vi "Prepare.vi"(8 "error in (no error)":errorcluster, 10 "Arguments":T1[](array[typedef]) {"Number" items=["? One or none"=0, "* Any"=-1, "+ At least one"=-2]}, 11 "LV Argument Parser in":refnum<class "LV Argument Parser.lvclass">) -> (0 "error out":errorcluster, 3 "LV Argument Parser out":refnum<class "LV Argument Parser.lvclass">)   [LabVIEW 2020, in "LV ArgParse.lvlib" / "LV Argument Parser.lvclass"]
uses:
  LV Argument Parser.lvclass
  Argument Definition.ctl
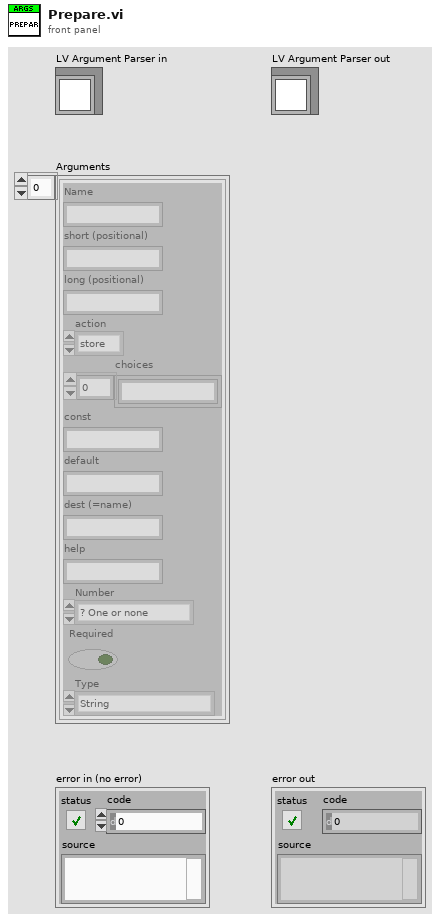
[diagram p1: front panel]
types:
  T1 = typedef "LV ArgParse.lvlib/LV Argument Parser.lvclass/Argument Definition.ctl" = cluster{"Name":string, "short (positional)":string, "long (positional)":string, "action":enum16{"store", "store-const", "store-false", "store-true", "append", "append-const", "count", "help", "version"}, "choices":string[], "const":string, "default":string, "dest (=name)":string, "help":string, "Number":i32, "Required":bool, "Type":enum16{"String", "Int", "UInt", "Float", "Bool", "Date", "Path"}}
  T2 = enum16{"store", "store-const", "store-false", "store-true", "append", "append-const", "count", "help", "version"}
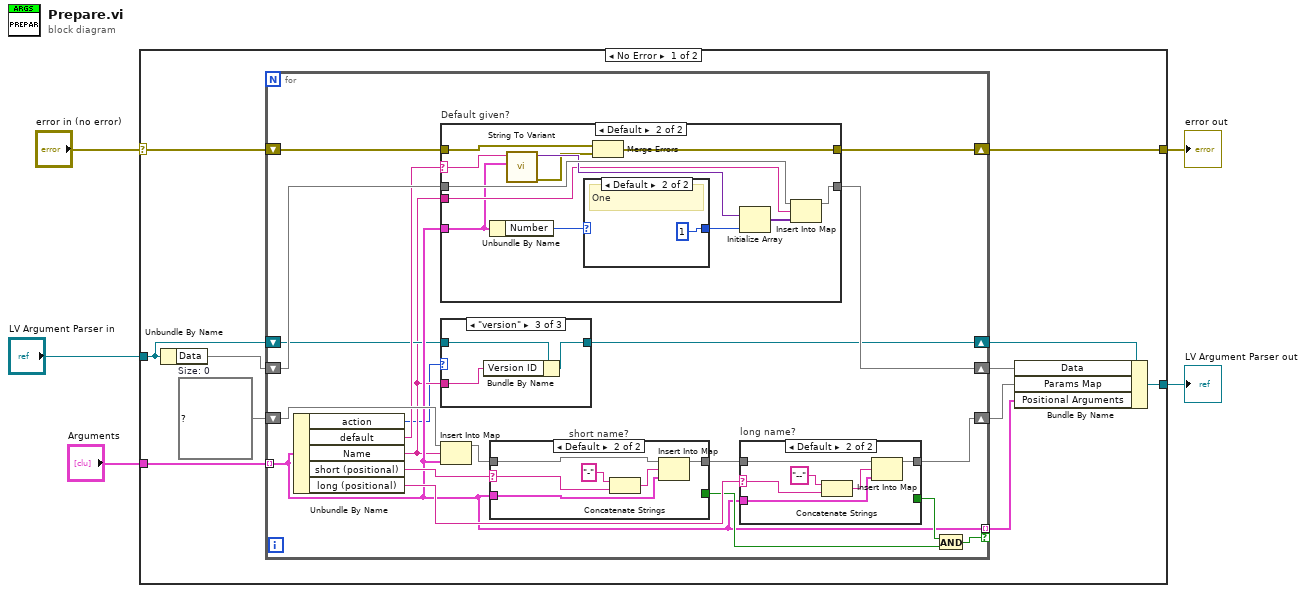
[diagram p0: block diagram]
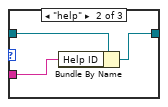
[diagram p3: hidden frame]
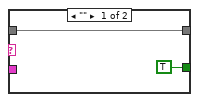
[diagram p6: hidden frame]
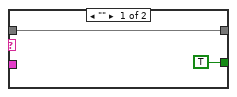
[diagram p7: hidden frame]
diagram:
  n1 = case shown="No Error" "error in (no error)" {
    selector: "error in (no error)" -> [w9 w75]
    tunnel: [w15 w76] -> w5
    tunnel: [w8 w75] -> w4
    tunnel: "LV Argument Parser in" -> [w6 w76]
    tunnel: "Arguments" -> [w12 _]
    frame No Error {
      w13 = map{string, T1} {}  # Size: 0
      n2 = Unbundle By Name(w6) -> ("Data"=w11:map{string, variant[]})
      n3 = for {
        tunnel: w12 -> [w23] mode=indexing
        tunnel: [w23] -> w16 mode=indexing if=w31
        shift-right: [w27] -> w14
        shift-left: w13 -> [w30]
        shift-right: [w25] -> w10
        shift-left: w11 -> [w26]
        shift-right: [w22] -> w8
        shift-left: w9 -> [w21]
        shift-right: [w19] -> w7
        shift-left: w6 -> [w20]
        n4 = Unbundle By Name(w23) -> ("action"=w17:T2, "default"=w24:string, "Name"=w18:string, "short (positional)"=w35:string, "long (positional)"=w34:string)
        n5 = case "Default given?" shown="Default" w24 {
          selector: w24 -> [_ w54]
          tunnel: w26 -> [w44 w56]
          tunnel: [w44 w55] -> w25
          tunnel: w23 -> [_ w47]
          tunnel: w18 -> [_ w51]
          tunnel: [w43 w49] -> w22
          tunnel: w21 -> [w43 w48]
          frame "" {
          }
          frame Default {
            n6 = Unbundle By Name(w47) -> ("Number"=w46:i32)
            n7 = call "String To Variant.vi"("Type"=w47, "String"=w54) -> ("error out"=w50:errorcluster, "Variant"=w53:variant)  [unwired: 8 in]
            n8 = case shown="Default" w46 {
              selector: w46 -> [w57 _]
              tunnel: [w57 1] -> w45
              frame 1.. {
                # "Defined Number"
              }
              frame Default {
                # "One"
              }
            }
            n9 = Merge Errors(w48, w50) -> (w49:errorcluster)
            n10 = Initialize Array(w53, w45) -> (w52:variant[])
            n11 = Insert Into Map(map in=w56, key=w51, value=w52) -> (map out=w55:map{string, variant[]})  [unwired: 2 out]
          }
        }
        n12 = case shown="\"version\"" w17 {
          tunnel: w20 -> [w36 w39 w42]
          tunnel: [w36 w38 w41] -> w19
          tunnel: w18 -> [_ w37 w40]
          frame Default {
          }
          frame "help" {
            n13 = Bundle By Name(cluster=w39, "Help ID"=w37) -> (w38:refnum<class "LV Argument Parser.lvclass">)
          }
          frame "version" {
            n14 = Bundle By Name(cluster=w42, "Version ID"=w40) -> (w41:refnum<class "LV Argument Parser.lvclass">)
          }
        }
        n15 = Insert Into Map(map in=w30, key=w18, value=w23) -> (map out=w29:map{string, T1})  [unwired: 2 out]
        n16 = case "short name?" shown="Default" w35 {
          selector: w35 -> [_ w72]
          tunnel: w29 -> [w68 w74]
          tunnel: [w68 w73] -> w28
          tunnel: w23 -> [_ w71]
          tunnel: [TRUE _] -> w33
          frame "" {
          }
          frame Default {
            n17 = Concatenate Strings("-" ("string"), w72) -> (w70:string)
            n18 = Insert Into Map(map in=w74, key=w70, value=w71) -> (map out=w73:map{string, T1})  [unwired: 2 out]
          }
        }
        n19 = case "long name?" shown="Default" w34 {
          selector: w34 -> [_ w64]
          tunnel: w28 -> [w60 w66]
          tunnel: [w60 w65] -> w27
          tunnel: w23 -> [_ w63]
          tunnel: [TRUE _] -> w32
          frame "" {
          }
          frame Default {
            n20 = Concatenate Strings("--" ("string"), w64) -> (w62:string)
            n21 = Insert Into Map(map in=w66, key=w62, value=w63) -> (map out=w65:map{string, T1})  [unwired: 2 out]
          }
        }
        n22 = And(x=w32, y=w33) -> (x .and. y?=w31:bool)
      }
      n23 = Bundle By Name(cluster=w7, "Data"=w10, "Params Map"=w14, "Positional Arguments"=w16) -> (w15:refnum<class "LV Argument Parser.lvclass">)
    }
    frame Error {
    }
  }
  "LV Argument Parser out" <- w5
  "error out" <- w4
